vi "Module Loop.vi"(8 "error in (no error)":errorcluster, 11 "Role Manager in":refnum<class "Role Manager.lvclass">) -> (0 "error out":errorcluster, 3 "Role Manager out":refnum<class "Role Manager.lvclass">)   [LabVIEW 2020, in "Volatus.lvlib" / "Role Manager.lvclass"]
uses:
  Role Manager.lvclass
  C:/dev/lv20CE/relink/lv-volatus/Volatus/Module/Module.lvclass
  Module/Module.lvclass
  Module/Module.lvclass/Module.ctl
  Role Manager.lvclass/Role Manager.ctl
  MessageQ/MessageQ.lvclass
  MessageQ/MessageQ.lvclass/MessageQ.ctl
  Module/Send to Self.vi
  MessageQ/Send.vi
  <vilib>/Utility/error.llb/Error Cluster From Error Code.vi
  lv-promises/Promises/Promise/Promise.lvclass
  Roles API/Roles API.lvclass
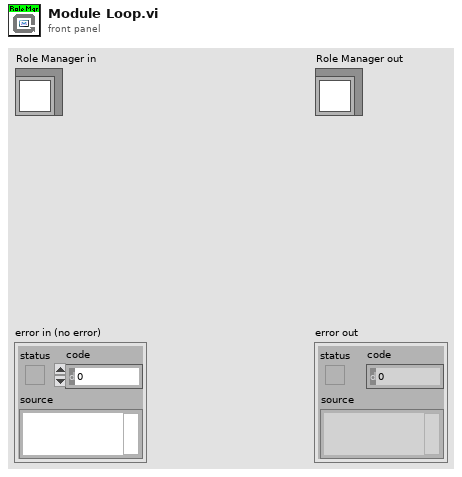
[diagram p1: front panel]
types:
  T1 = enum32{"Invalid", "Standard", "Closed", "Hidden", "Minimized", "Maximized"}
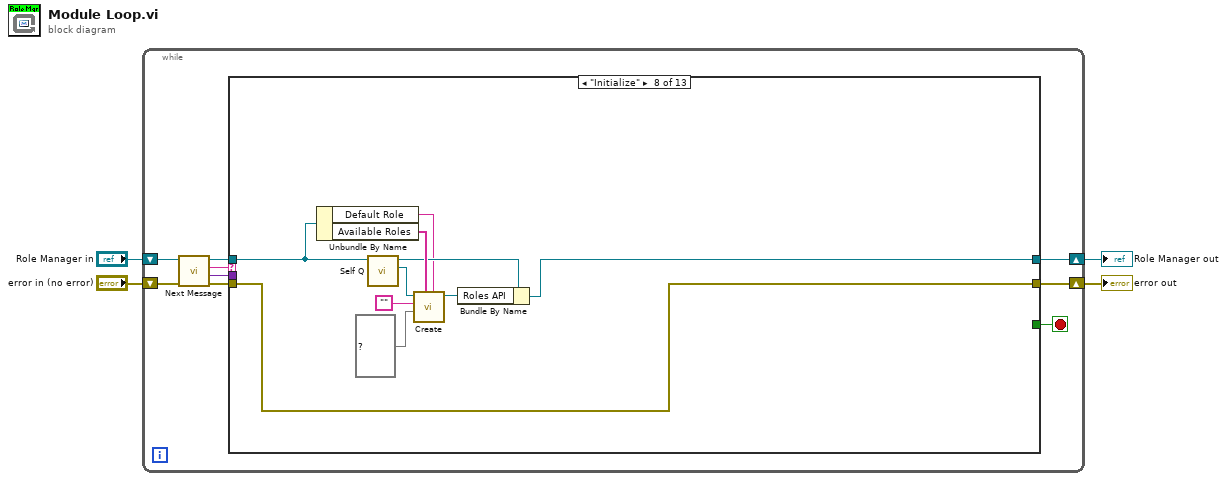
[diagram p0: block diagram]
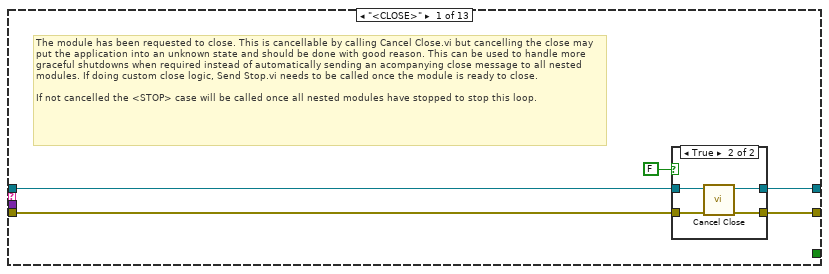
[diagram p2: hidden frame]
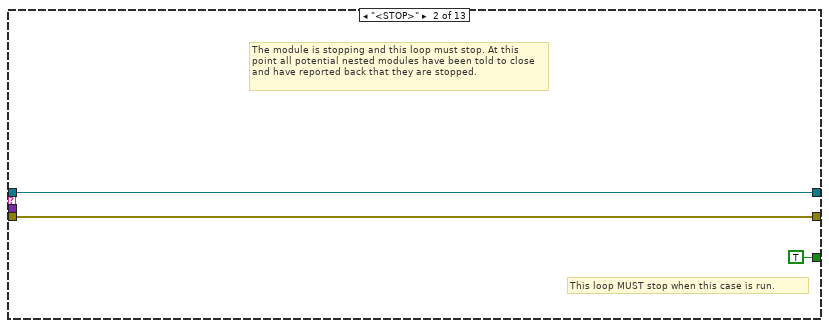
[diagram p4: hidden frame]
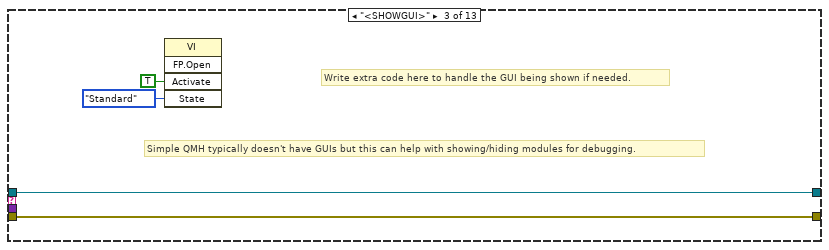
[diagram p5: hidden frame]
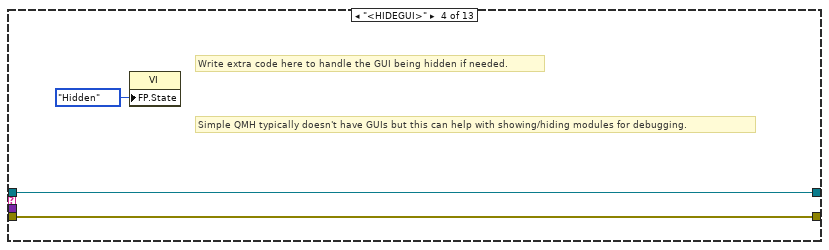
[diagram p6: hidden frame]
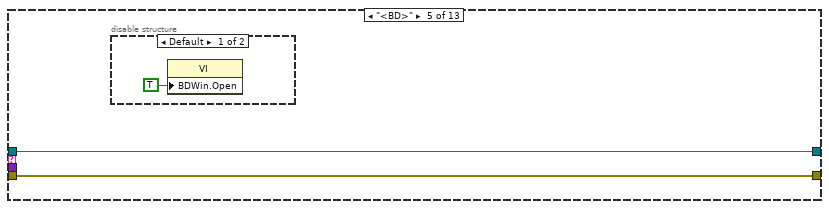
[diagram p7: hidden frame]
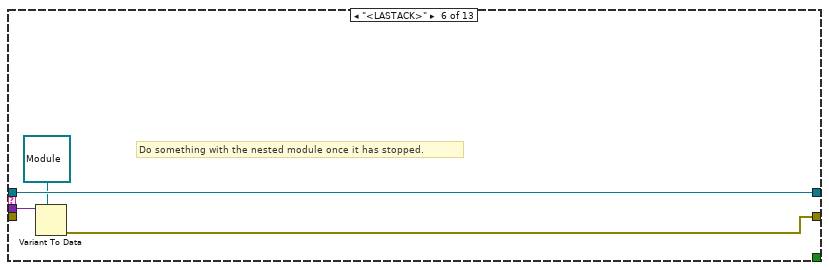
[diagram p9: hidden frame]
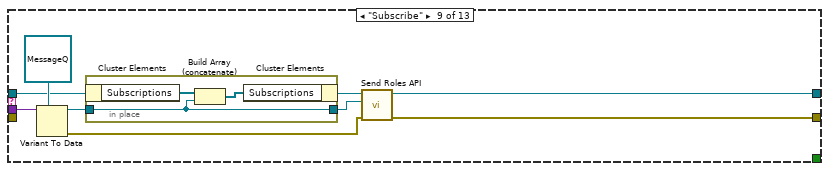
[diagram p11: hidden frame]
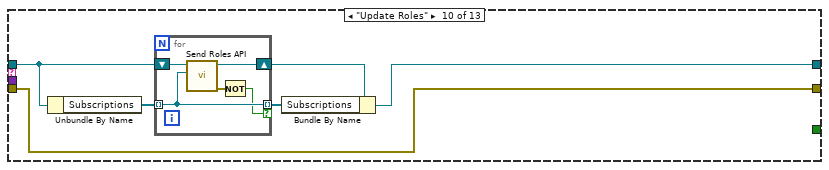
[diagram p12: hidden frame]
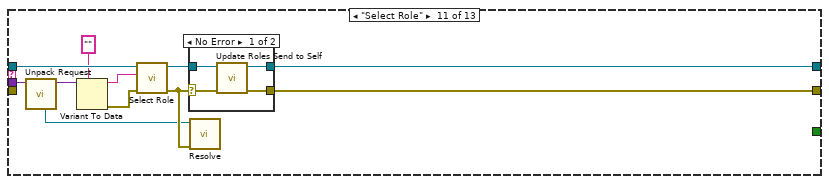
[diagram p13: hidden frame]
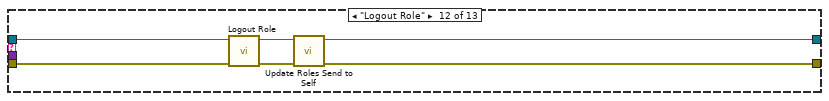
[diagram p15: hidden frame]
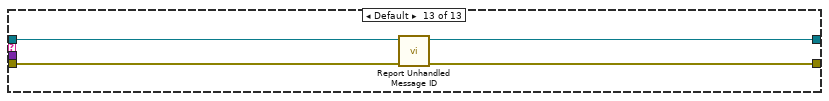
[diagram p16: hidden frame]
diagram:
  n1 = while {
    shift-right: [w8] -> w1
    shift-left: "Role Manager in" -> [w13]
    shift-right: [w5] -> w2
    shift-left: "error in (no error)" -> [w12]
    stop <- w7 stop-if-true
    n2 = call "Next Message.vi"("error in (no error)"=w12, "Module in"=w13) -> ("error out"=w11:errorcluster, "Data"=w6:variant, "ID"=w10:string, "Module out"=w9:refnum<class "Role Manager.lvclass">)  [unwired: 6 in]
    n3 = case shown="\"Initialize\"" w10 {
      tunnel: w11 -> [w18 w26 w30 w33 w35 _ w42 w45 _ w66 _ w99 w103]
      tunnel: w9 -> [w16 w27 w31 w34 w36 w41 w43 w50 w60 w70 w86 w97 w101]
      tunnel: [w15 w27 w31 w34 w36 w41 w43 w48 w54 w67 w77 w94 w100] -> w8
      tunnel: [_ TRUE _ _ _ _ _ _ _ _ _ _ _] -> w7
      tunnel: w6 -> [_ _ _ _ _ w40 _ _ w62 _ w84 _ _]
      tunnel: [w17 w26 w30 w33 w35 w38 w42 w45 w55 w66 w79 w96 w102] -> w5
      frame "<CLOSE>" {
        # "The module has been requested to close. This is cancellable by calling Cancel Close.vi but cancelling the close may put the application into an unknown state and should be done with good reason. This can be used to handle more graceful shutdowns when required instead of automatically sending an acompanying close message to all nested modules. If doing custom close logic, Send Stop.vi needs to be called once the module is ready to close.\n\nIf not cancelled the <STOP> case will be called once all nested modules have stopped to stop this loop."
        n4 = case shown="True" FALSE {
          tunnel: w18 -> [w19 w24]
          tunnel: [w19 w23] -> w17
          tunnel: w16 -> [w20 w22]
          tunnel: [w20 w21] -> w15
          frame False {
          }
          frame True {
            n5 = call "Cancel Close.vi"("error in (no error)"=w24, "Module in"=w22) -> ("error out"=w23:errorcluster, "Module out"=w21:refnum<class "Role Manager.lvclass">)  [unwired: 8 in]
          }
        }
      }
      frame "<STOP>" {
        # "This loop MUST stop when this case is run."
        # "The module is stopping and this loop must stop. At this point all potential nested modules have been told to close and have reported back that they are stopped."
      }
      frame "<SHOWGUI>" {
        # "Simple QMH typically doesn't have GUIs but this can help with showing/hiding modules for debugging."
        # "Write extra code here to handle the GUI being shown if needed."
        n6 = invoke class="VI" method="FP.Open"("Activate"=TRUE ("Activate?"), "State"=T1."Standard") -> ()  [unwired: 3 in, 5 out]
      }
      frame "<HIDEGUI>" {
        # "Simple QMH typically doesn't have GUIs but this can help with showing/hiding modules for debugging."
        # "Write extra code here to handle the GUI being hidden if needed."
        n7 = property class="VI"("FP.State"=T1."Hidden" ("Front Panel Window:State")) -> ()  [unwired: 2 in, 2 out]
      }
      frame "<BD>" {
        n8 = disable-structure shown="Default" {
          frame condition #0 (active) {
            n9 = property class="VI"("BDWin.Open"=TRUE ("Block Diagram Window:Open")) -> ()  [unwired: 2 in, 2 out]
          }
          frame condition #1 {
          }
        }
      }
      frame "<LASTACK>" {
        # "Do something with the nested module once it has stopped."
        n10 = Variant To Data(type=refnum<class "Module.lvclass"> refnum ("Volatus:Module"), Variant=w40) -> (error out=w38:errorcluster)  [unwired: 1 in, 1 out]
      }
      frame "<TIMEOUT>" {
        # "No message for this module was received in time"
      }
      frame "Initialize" {
        n11 = Unbundle By Name(w50) -> ("Default Role"=w44:string, "Available Roles"=w53:string[])
        n12 = call "Self Q.vi"("Module in"=w50) -> ("Self Q"=w52:refnum<class "MessageQ.lvclass">, "Module out"=w49:refnum<class "Role Manager.lvclass">)  [unwired: 9 in]
        n13 = call "Create.vi"("Default Role"=w44, "Available"=w53, "Effective Roles"=set{string} {}, "Current Role"="", "Manager"=w52) -> ("Roles API out"=w51:refnum<class "Roles API.lvclass">)  [unwired: 5 in, 1 out]
        n14 = Bundle By Name(cluster=w49, "Roles API"=w51) -> (w48:refnum<class "Role Manager.lvclass">)
      }
      frame "Subscribe" {
        n15 = Variant To Data(type=refnum<class "MessageQ.lvclass"> refnum ("Volatus:MessageQ"), Variant=w62) -> (data=w59:refnum<class "MessageQ.lvclass">, error out=w56:errorcluster)  [unwired: 1 in]
        n16 = in-place {
          in-place-border: w59 -> [w63]
          in-place-border: [w63] -> w57
          n17 = in-place-cluster #1(w60) -> ("Subscriptions"=w65:refnum<class "MessageQ.lvclass">[])
          n18 = Build Array (concatenate)(w65, w63) -> (w64:refnum<class "MessageQ.lvclass">[])
          n19 = in-place-cluster #1("Subscriptions"=w64) -> (w58:refnum<class "Role Manager.lvclass">)
        }
        n20 = call "Send Roles API.vi"("error in (no error)"=w56, "Subscriber"=w57, "Role Manager in"=w58) -> ("error out"=w55:errorcluster, "Role Manager out"=w54:refnum<class "Role Manager.lvclass">)  [unwired: 7 in]
      }
      frame "Update Roles" {
        n21 = Unbundle By Name(w70) -> ("Subscriptions"=w69:refnum<class "MessageQ.lvclass">[])
        n22 = for {
          shift-right: [w72] -> w71
          shift-left: w70 -> [w76]
          tunnel: w69 -> [w75] mode=indexing
          tunnel: [w75] -> w68 mode=indexing if=w73
          n23 = call "Send Roles API.vi"("Subscriber"=w75, "Role Manager in"=w76) -> ("error out"=w74:errorcluster, "Role Manager out"=w72:refnum<class "Role Manager.lvclass">)  [unwired: 8 in]
          n24 = Not(x=w74) -> (.not. x?=w73:bool)
        }
        n25 = Bundle By Name(cluster=w71, "Subscriptions"=w68) -> (w67:refnum<class "Role Manager.lvclass">)
      }
      frame "Select Role" {
        n26 = call "Unpack Request.vi"("Request Data"=w84) -> ("Data"=w83:variant, "Promise"=w80:refnum<class "Promise.lvclass">)  [unwired: 8 in, 1 out]
        n27 = Variant To Data(type="", Variant=w83) -> (data=w82:string, error out=w81:errorcluster)  [unwired: 1 in]
        n28 = call "Select Role.vi"("error in (no error)"=w81, "Role"=w82, "Role Manager in"=w86) -> ("error out"=w87:errorcluster, "Role Manager out"=w78:refnum<class "Role Manager.lvclass">)  [unwired: 7 in]
        n29 = case shown="No Error" w87 {
          selector: w87 -> [w91 w92]
          tunnel: [w90 w92] -> w79
          tunnel: w78 -> [w89 w93]
          tunnel: [w88 w93] -> w77
          frame No Error {
            n30 = call "Update Roles Send to Self.vi"("error in (no error)"=w91, "Role Manager in"=w89) -> ("error out"=w90:errorcluster, "Role Manager out"=w88:refnum<class "Role Manager.lvclass">)  [unwired: 8 in]
          }
          frame Error {
          }
        }
        n31 = call "Resolve.vi"("error in (no error)"=w87, "Promise in"=w80) -> ()  [unwired: 8 in, 2 out]
      }
      frame "Logout Role" {
        n32 = call "Logout Role.vi"("error in (no error)"=w99, "Role Manager in"=w97) -> ("error out"=w98:errorcluster, "Role Manager out"=w95:refnum<class "Role Manager.lvclass">)  [unwired: 8 in]
        n33 = call "Update Roles Send to Self.vi"("error in (no error)"=w98, "Role Manager in"=w95) -> ("error out"=w96:errorcluster, "Role Manager out"=w94:refnum<class "Role Manager.lvclass">)  [unwired: 8 in]
      }
      frame Default {
        n34 = call "Report Unhandled Message ID.vi"("error in (no error)"=w103, "Module in"=w101) -> ("error out"=w102:errorcluster, "Module out"=w100:refnum<class "Role Manager.lvclass">)  [unwired: 8 in]
      }
    }
  }
  "error out" <- w2
  "Role Manager out" <- w1
